vi "Create Delete Array.vi"   [LabVIEW 2012, in "Scripting Tools.lvlib"]
uses:
  Scripting Tools.lvlib
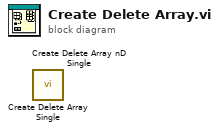
[diagram p0: block diagram]
diagram:
  n1 = call "Create Delete Array Single.vi"() -> ()  [unwired: 8 in, 4 out]
  n2 = call "Create Delete Array nD Single.vi"() -> ()  [unwired: 8 in, 4 out]
